vi "RemoteVI Apply Modifiers.vi"(0 "mods":u8, 5 "mods set":u8, 7 "popup":bool, 8 "hWnd":u64, 11 "error in":errorcluster) -> (4 "mods set out":u8, 15 "error out":errorcluster)   [LabVIEW 2020, in "RemoteVI.lvlib"]
doc: "Brings the modifier keys LabVIEW sees in line with the ones the remote user holds. When mods differs from mods set (what was last written) and no LabVIEW popup is open, mods is written into the key state of the UI thread that owns hWnd with RemoteVI Write Modifiers.vi (this LabVIEW's, or another LabVIEW's over VI Server) and mods set out becomes mods; otherwise nothing is written and mods set passes through, so a change made while a popup is open is written with the first message after it closes. A popup's modal loop holds the UI thread, and Set Modifier Keys.vi runs in it, so it would block until the popup closes. Mouse tracking does not block it (measured). An incoming error skips the write."
uses:
  RemoteVI.lvlib
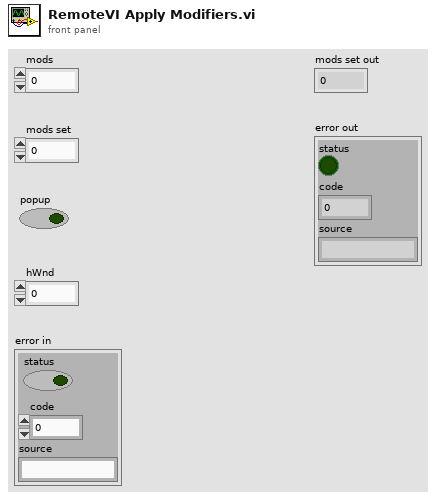
[diagram p1: front panel]
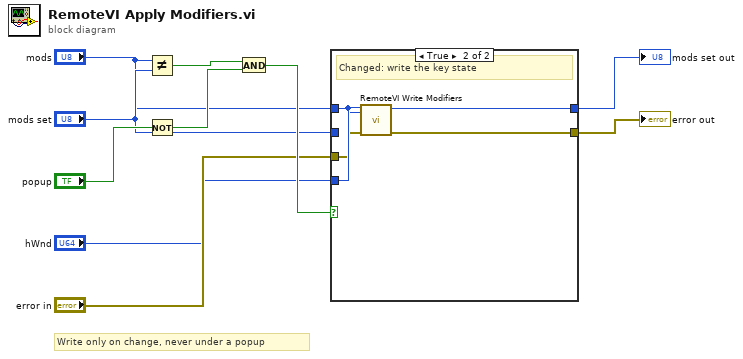
[diagram p0: block diagram]
diagram:
  # "Write only on change, never under a popup"
  n1 = Not Equal?(x="mods", y="mods set") -> (x != y?=w6:bool)
  n2 = Not(x="popup") -> (.not. x?=w7:bool)
  n3 = And(x=w6, y=w7) -> (x .and. y?=w8:bool)
  n4 = case shown="True" w8 {
    tunnel: "mods" -> [_ w13]
    tunnel: "mods set" -> [w11 _]
    tunnel: "error in" -> [w12 w14]
    tunnel: "hWnd" -> [_ w15]
    tunnel: [w11 w13] -> w9
    tunnel: [w12 w16] -> w10
    frame False {
      # "Unchanged, or a popup holds the UI thread"
    }
    frame True {
      # "Changed: write the key state"
      n5 = call "RemoteVI Write Modifiers.vi"("hWnd"=w15, "mods"=w13, "error in"=w14) -> ("error out"=w16:errorcluster)  [unwired: 12 in]
    }
  }
  "mods set out" <- w9
  "error out" <- w10
